vi "Servo_Control_Ex.vi"() -> ()   [LabVIEW 2026]
panel:
  in  "Angulo":u8 max=180 format="%x"
  in  "Canal":u8
  out "respuesta":string
  in  "VISA resource name":refnum<visa-resource-name>
  in  "Stop Button":bool
  out "error out":errorcluster
  # "Ejemplo: Servomotor"
  # "Descripción: controla un servomotor segun su canal y angulo"
  # "Configuracion"
  # "Indicadores"
  # "Control"
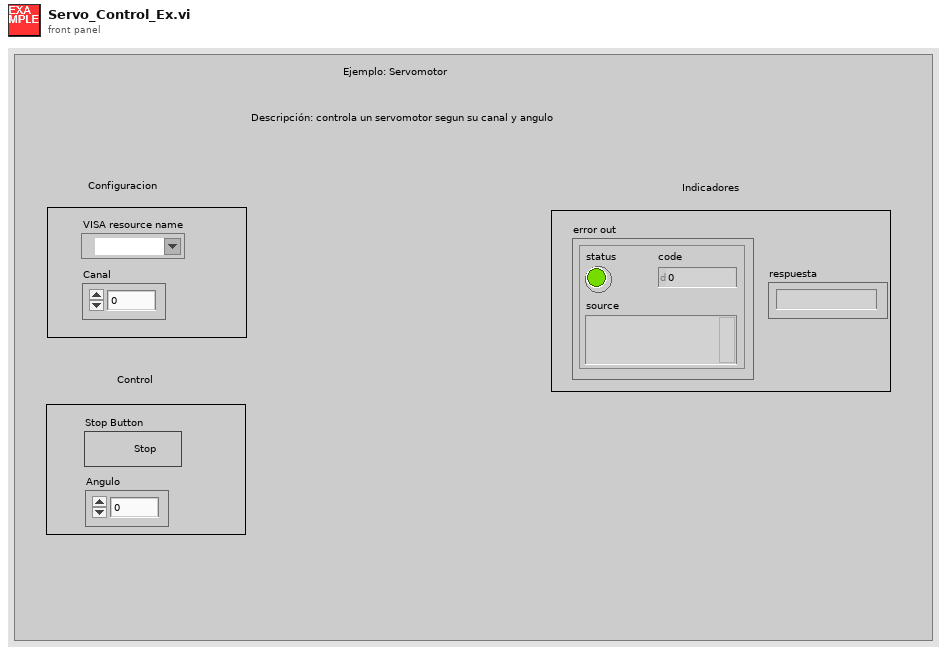
[diagram p1: front panel]
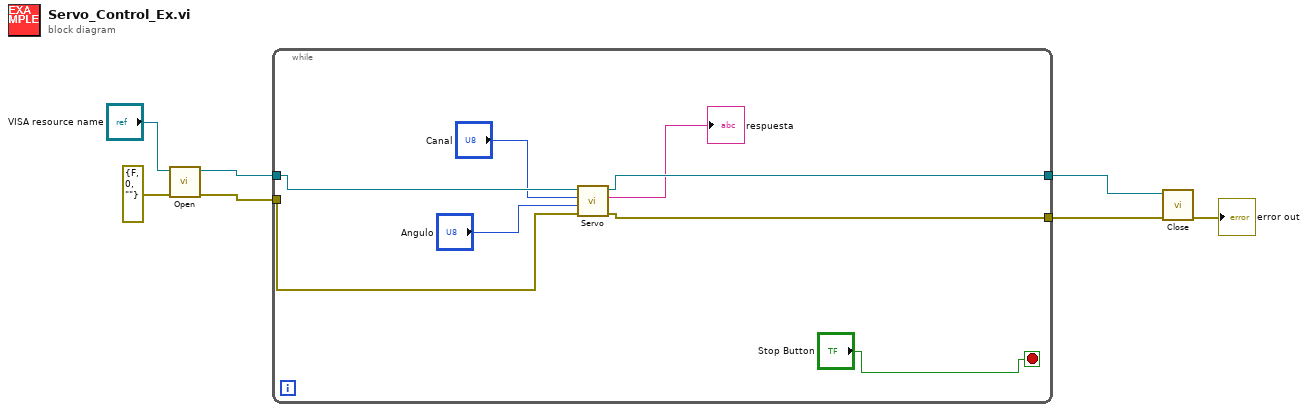
[diagram p0: block diagram]
diagram:
  n1 = call "Open.vi"("error in (no error)"=errorcluster {"status"=FALSE, "code"=0, "source"=""}, "VISA resource name"="VISA resource name") -> ("error out"=w7:errorcluster, "VISA resource name out"=w6:refnum<visa-resource-name>)  [unwired: 8 in]
  n2 = while {
    tunnel: w6 -> [w14]
    tunnel: w7 -> [w13]
    tunnel: [w12] -> w2
    tunnel: [w11] -> w1
    stop <- "Stop Button" stop-if-true
    n3 = call "Servo.vi"("error in (no error)"=w13, "Angulo"="Angulo", "Canal"="Canal", "VISA resource name"=w14) -> ("error out"=w11:errorcluster, "respuesta"=→"respuesta":string, "VISA resource name out"=w12:refnum<visa-resource-name>)  [unwired: 5 in]
  }
  n4 = call "Close.vi"("error in (no error)"=w1, "VISA resource name"=w2) -> ("error out"=→"error out":errorcluster)  [unwired: 9 in]
